vi "Values update in report.vi"(6 "MESURED  Voltage":string, 7 "array":string[][](array[string]), 8 "MESURED":string, 9 "HI SET":string, 10 "LO SET":string, 11 "Voltage":string) -> (3 "output array":string[][](array[string]))   [LabVIEW 2021]
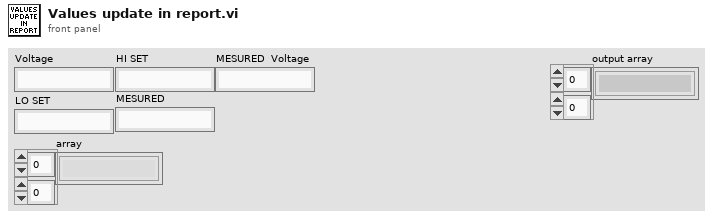
[diagram p1: front panel]
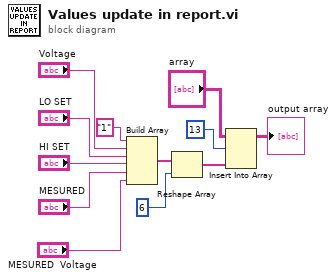
[diagram p0: block diagram]
diagram:
  n1 = Build Array("1" ("new element/subarray"), "Voltage", "LO SET", "HI SET", "MESURED", "MESURED  Voltage") -> (w4:string[])
  n2 = Reshape Array(w4, 6 ("dimension size")) -> (w3:string[])
  n3 = Insert Into Array(array="array", index (row)=13 ("index"), new element=w3) -> (→"output array":string[][])  [unwired: 1 in]
